vi "configuration UI.vi"() -> ()   [LabVIEW 2013, in "CVT editor node.lvclass"]
uses:
  CVT editor node.lvclass
  <vilib>/NI/Configuration Framework/Node/NodeRef.ctl
  <vilib>/NI/Configuration Framework/Node/NISE_CEF_Node.lvclass
  <vilib>/NI/AMC/Message Queue.ctl
  <vilib>/NI/AMC/Message.ctl
  <vilib>/NI/Tools/Keyed Array/KeyedArray.ctl
  <vilib>/NI/Configuration Framework/Node/UserEventRef.ctl
  <vilib>/NI/Configuration Framework/Controls/EventCluster.ctl
  <vilib>/NI/DCAF UI Toolkit/Controls/Move One Left.ctl
  <vilib>/NI/DCAF UI Toolkit/Controls/Move One Right.ctl
  <vilib>/Utility/miscctls.llb/LVPositionTypeDef.ctl
  <vilib>/Utility/miscctls.llb/LVRowAndColumnTypeDef.ctl
  CVT editor node.lvclass/CVT editor node.ctl
  configuration/CVT configuration.lvclass/CVT configuration.ctl
  <vilib>/NI/Tag Bus Module Framework/channel/channel classification.ctl
  <vilib>/NI/Tag Bus/tag/Data Type.ctl
  <vilib>/NI/Configuration Framework/serializable configuration/NISE_CEF_serializable configuration.lvclass/NISE_CEF_serializable configuration.ctl
  configuration/CVT configuration.lvclass
  <vilib>/NI/Tag Bus/tag/tag descriptor.lvclass/tag descriptor.ctl
  configuration/Write Create Tags_.vi
  <vilib>/Utility/LVClass/Get LV Class Name.vi
  <vilib>/NI/Configuration Framework/error generator/NISE_error generator.vi
  Item Names.vi
  Apply Filter_1D.vi
  Apply Filter_2D.vi
  <vilib>/NI/Module Execution Interface/Engine Configuration/engine configuration.lvclass
  <vilib>/NI/DCAF/Tag Editor Core/Configuration Editor/Classes/Module editor node/module editor node.lvclass
  <vilib>/NI/Configuration Framework/NISE_CEF_TreeControl.lvlib
  <vilib>/NI/Tag Bus/tag/tag descriptor.lvclass
  <vilib>/NI/Tag Bus Module Framework/channel/TBM channel.lvclass
  <vilib>/NI/DCAF/Tag Editor Core/Configuration Editor/Classes/Engine Parent/Engine Parent Editor Node.lvclass
  <vilib>/NI/Configuration Framework/serializable configuration/NISE_CEF_serializable configuration.lvclass
  <vilib>/NI/DCAF UI Toolkit/Controls/DCAF UI Elements.lvlib
  <vilib>/NI/Tools/Keyed Array/Tools_KeyedArray.lvlib
  <vilib>/NI/AMC/AMC.lvlib
panel:
  in  "Top Level Tab Control":enum32{"CVT Channel Mappings"}(tab)
  in  "Create Tags?":bool=TRUE
  in  "Filter":string
  in  "add to":T1
  in  "remove to":T2
  in  "add from":T1
  in  "remove from":T2
  in  "to CVT List":i32(listbox)
  in  "from CVT List":i32(listbox)
  in  "avail tags":i32(listbox)
  in  "Direction":enum32{"From CVT", "To CVT"}(radio)
  in  "user event":T3
  in  "main queue":T4
  in  "node ref":T5
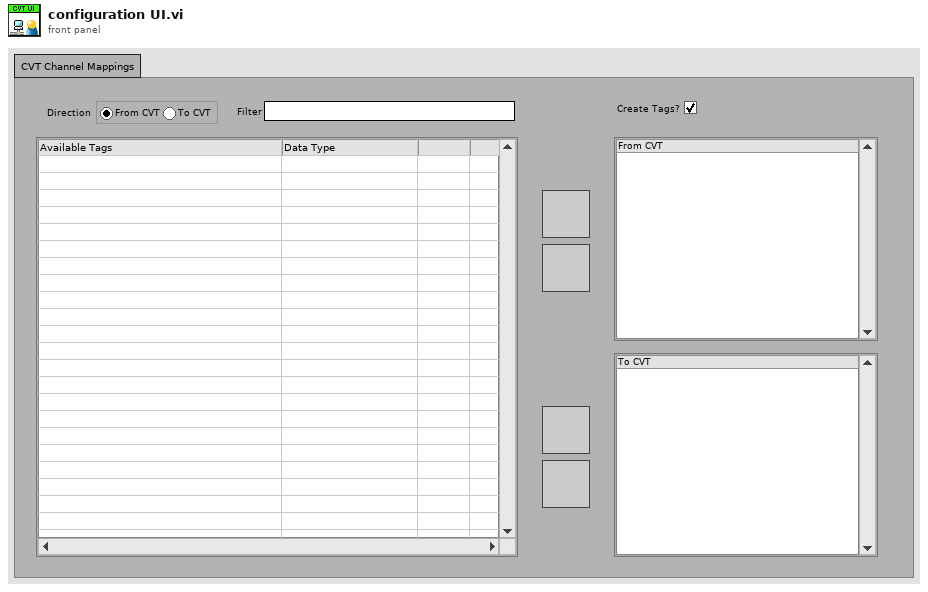
[diagram p1: front panel]
types:
  T1 = typedef "DCAF UI Elements.lvlib/Move One Right.ctl" = bool
  T2 = typedef "DCAF UI Elements.lvlib/Move One Left.ctl" = bool
  T3 = typedef "NISE_CEF_Node.lvclass/UserEventRef.ctl" = refnum<user-event>
  T4 = typedef "AMC.lvlib/Message Queue.ctl" = refnum<queue>
  T5 = typedef "NISE_CEF_Node.lvclass/NodeRef.ctl" = refnum<data-value>
  T6 = typedef "LVPositionTypeDef.ctl" = cluster{"Left":i32, "Top":i32}
  T7 = typedef "NISE_CEF_TreeControl.lvlib/EventCluster.ctl" = cluster{"command":string, "data":string}
  T8 = typedef "LVRowAndColumnTypeDef.ctl" = cluster{"Row":i32, "Column":i32}
  T9 = enum8{"Enabled", "Disabled", "Disabled and Grayed Out"}
  T10 = typedef "tag bus.lvlib/tag descriptor.lvclass/Data Type.ctl" = enum16{"Double", "Single", "I64", "I32", "I16", "I8", "U64", "U32", "U16", "U8", "Boolean", "String", "Array of Double", "Array of Single", "Array of I64", "Array of I32", "Array of I16", "Array of I8", "Array of U64", "Array of U32", "Array of U16", "Array of U8", "Array of Boolean", "Array of String"}
  T11 = typedef "TBM channel.lvclass/channel classification.ctl" = enum16{"input data", "output data", "processing parameter", "processing result"}
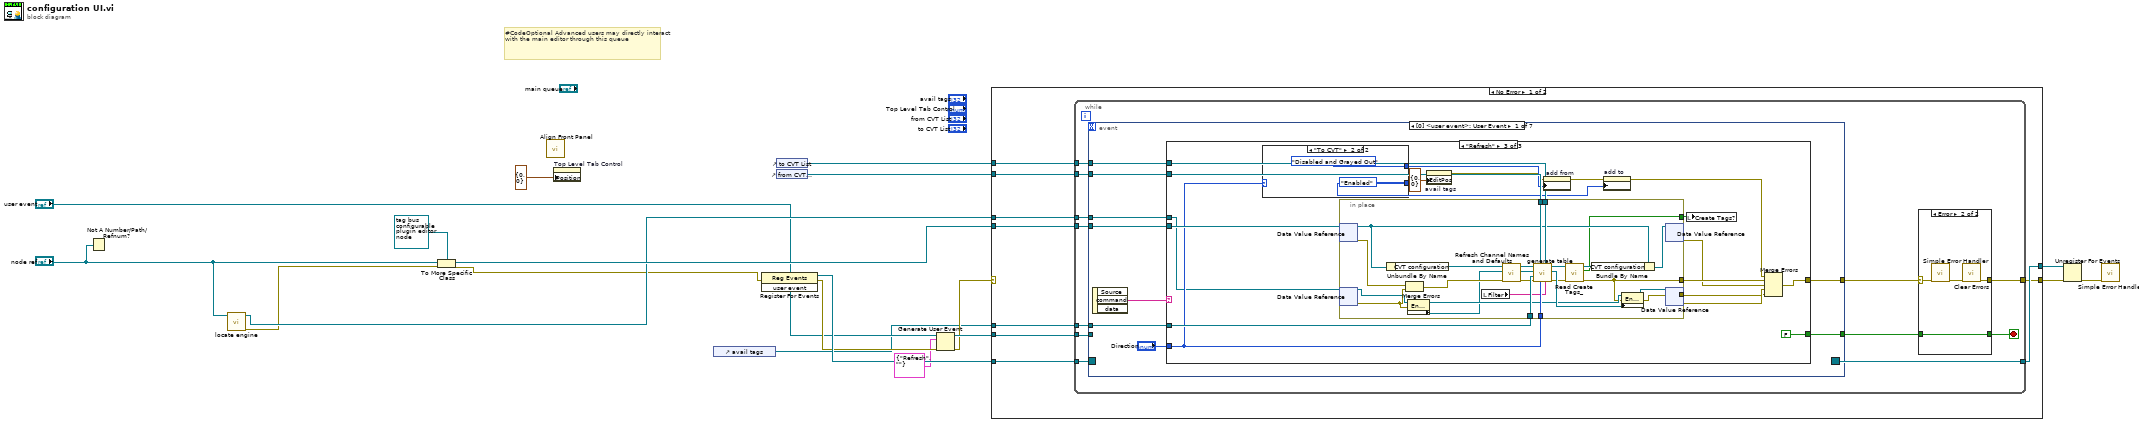
[diagram p0: block diagram]
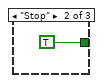
[diagram p4: hidden frame]
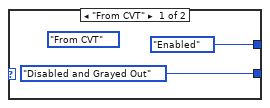
[diagram p5: hidden frame]
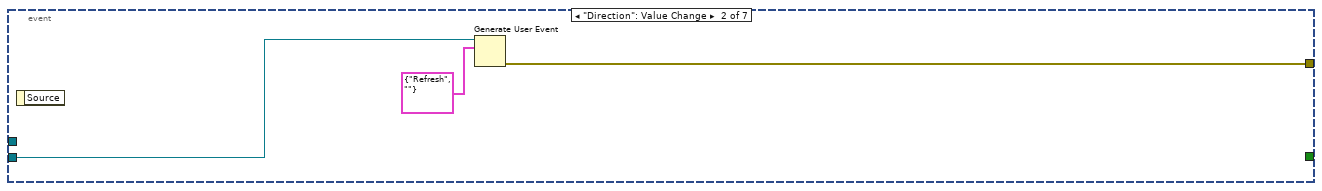
[diagram p6: hidden frame]
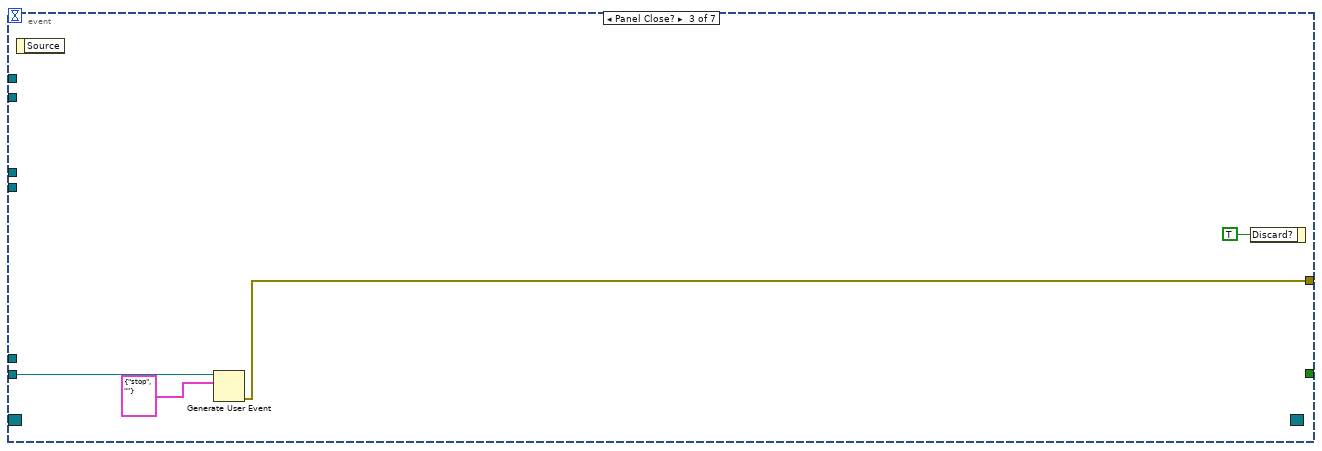
[diagram p7: hidden frame]
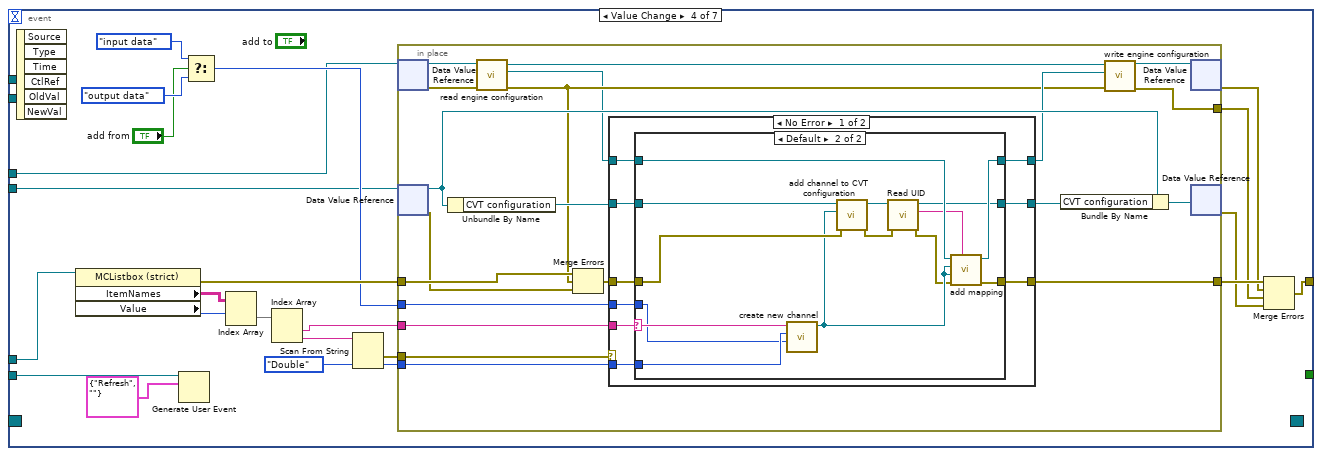
[diagram p8: hidden frame]
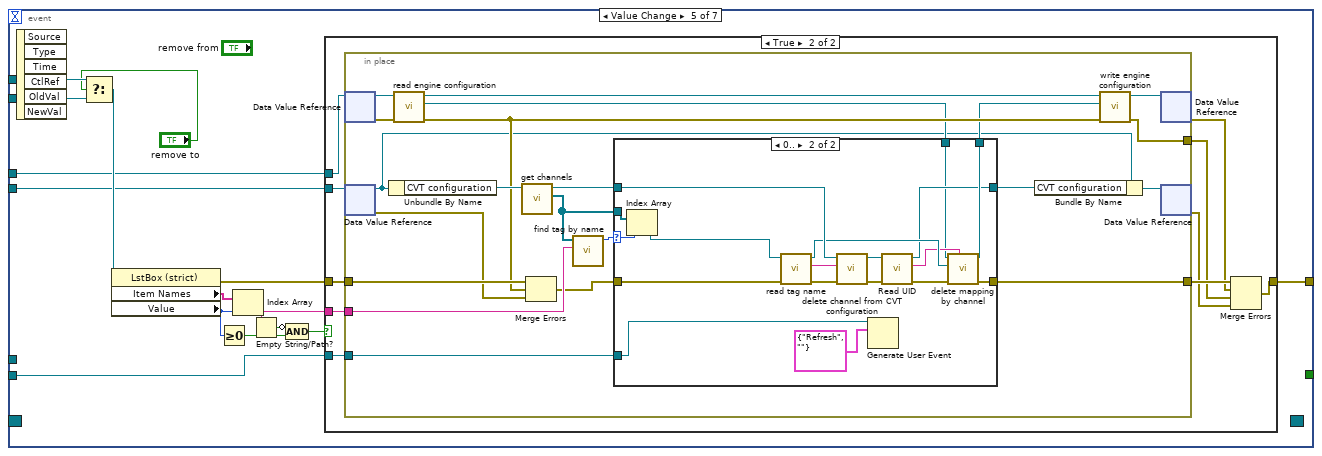
[diagram p11: hidden frame]
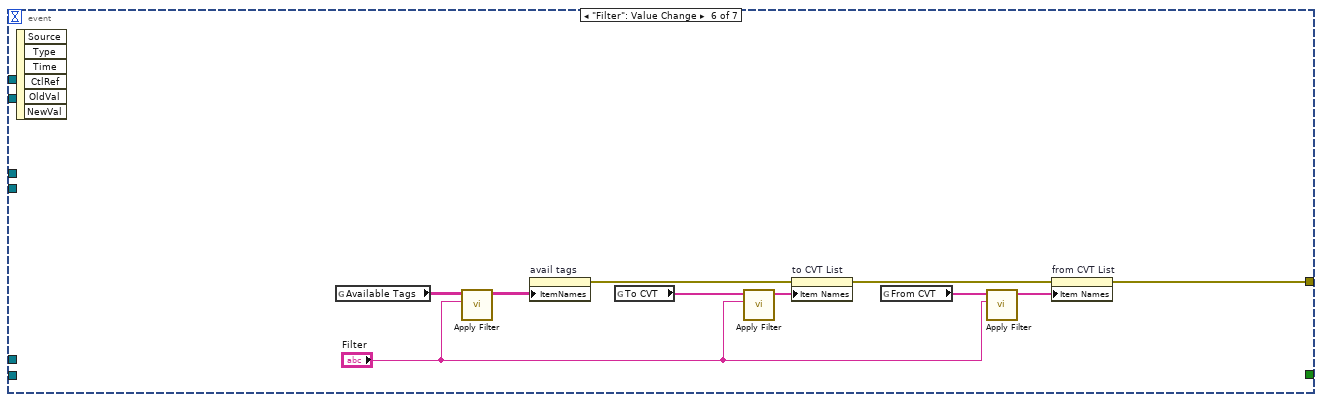
[diagram p14: hidden frame]
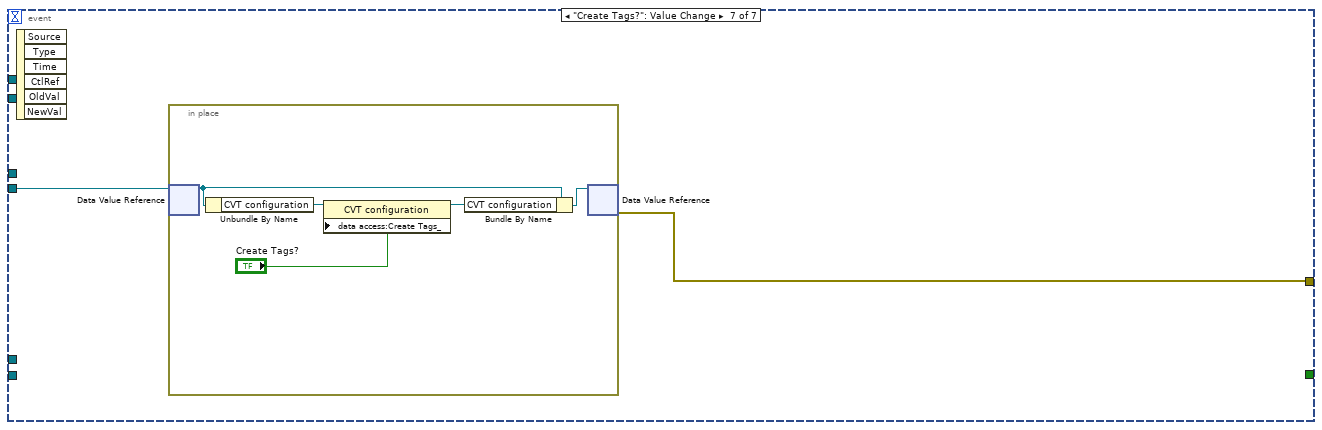
[diagram p15: hidden frame]
diagram:
  # "#CodeOptional Advanced users may directly interact with the main editor through this queue"
  n1 = Not A Number/Path/Refnum?(number/path/refnum="node ref") -> ()  [unwired: 1 out]
  n2 = call <vilib>:"locate engine.vi"("component"="node ref") -> ("error out"=w6:errorcluster, "engine"=w13:refnum<data-value>)  [unwired: 9 in]
  n3 = To More Specific Class(target class=refnum<data-value> refnum ("data value reference"), reference="node ref", error in=w6) -> (specific class reference=w15:refnum<data-value>, error out=w1:errorcluster)
  n4 = call <vilib>:"Align Front Panel.vi"() -> ()  [unwired: 10 in, 2 out]
  n5 = property on="Top Level Tab Control" class="TabCtl (strict)"("Position"=T6 {"Left"=0, "Top"=0}) -> ()  [unwired: 2 in, 2 out]
  n6 = control-ref of="avail tags"() -> (w2:refnum<vi>)
  n7 = register-events(error in=w1, "user event") -> (reference out=w19:refnum<event-registration>, error out=w12:errorcluster)  [unwired: 1 in]
  n8 = control-ref of="to CVT List"() -> (w4:refnum<vi>)
  n9 = control-ref of="from CVT List"() -> (w3:refnum<vi>)
  n10 = Generate User Event(user event="user event", event data cluster=T7 {"command"="Refresh", "data"=""} ("event data"), error in=w12) -> (user event out=w10:T3, error out=w8:errorcluster)  [unwired: 1 in]
  n11 = case shown="No Error" w8 {
    selector: w8 -> [_ w270]
    tunnel: w19 -> [w28 w269]
    tunnel: [w27 w269] -> w18
    tunnel: [w26 w270] -> w17
    tunnel: w15 -> [w25 _]
    tunnel: w13 -> [w24 _]
    tunnel: w2 -> [w23 _]
    tunnel: w4 -> [w22 _]
    tunnel: w3 -> [w21 _]
    tunnel: w10 -> [w20 _]
    frame No Error {
      n12 = while {
        tunnel: w28 -> [w40]
        tunnel: [w39] -> w27
        tunnel: w25 -> [w34]
        tunnel: w24 -> [w33]
        tunnel: w20 -> [w32]
        tunnel: w23 -> [w31]
        tunnel: w22 -> [w30]
        tunnel: w21 -> [w29]
        tunnel: [w35] -> w26
        stop <- w37 stop-if-true
        n13 = event shown="[0] <user event>: User Event" {
          selector: w40 -> [_ _ _ _ _ _ _]
          dyn-events: [_ _ _ _ _ _ _] -> w39
          timeout: _ -> [_ _ _ _ _ _ _]
          tunnel: [w55 _ _ _ _ _ _] -> w36
          tunnel: [w53 w105 w108 w118 w189 w261 w262] -> w38
          tunnel: w34 -> [w52 _ _ w114 w186 _ w263]
          tunnel: w33 -> [w51 _ _ w115 w185 _ _]
          tunnel: w32 -> [_ w106 w109 w133 w188 _ _]
          tunnel: w31 -> [w50 _ _ w128 _ _ _]
          tunnel: w30 -> [w49 _ _ _ w197 _ _]
          tunnel: w29 -> [w48 _ _ _ w198 _ _]
          event User Event {
            n14 = event-data() -> ("command"=w54:string)  [unwired: 1 in, 2 out]
            n15 = case shown="\"Refresh\"" w54 {
              tunnel: [_ TRUE FALSE] -> w55
              tunnel: [_ _ w69] -> w53
              tunnel: w52 -> [_ _ w70]
              tunnel: w51 -> [_ _ w60]
              tunnel: w50 -> [_ _ w73]
              tunnel: w49 -> [_ _ w72]
              tunnel: w48 -> [_ _ w71]
              tunnel: "Direction" -> [_ _ w62]
              frame Default {
              }
              frame "Stop" {
              }
              frame "Refresh" {
                n16 = case shown="\"To CVT\"" w62 {
                  tunnel: [T9."Enabled" ("Disabled") T9."Disabled and Grayed Out" ("Disabled")] -> w66
                  tunnel: [T9."Disabled and Grayed Out" ("Disabled") T9."Enabled" ("Disabled")] -> w65
                  frame "From CVT" {
                    (unwired) enum32{"From CVT", "To CVT"}."From CVT" ("Direction")
                  }
                  frame "To CVT" {
                  }
                }
                n17 = in-place {
                  in-place-border: [w81] -> w74
                  in-place-border: w73 -> [w104]
                  in-place-border: w72 -> [w103]
                  in-place-border: w71 -> [w102]
                  in-place-border: w62 -> [w101]
                  in-place-border: [w93] -> w58
                  in-place-border: [w80] -> w57
                  n18 = in-place-dvr #1(w70) -> (w99:refnum<class "CVT editor node.lvclass">, w100:errorcluster)
                  n19 = in-place-dvr #2(w60) -> (w96:refnum<class "Engine Parent Editor Node.lvclass">, w97:errorcluster)
                  n20 = Unbundle By Name(w99) -> ("CVT configuration"=w89:refnum<class "CVT configuration.lvclass">)
                  n21 = Merge Errors(w100, w97) -> (w91:errorcluster)
                  n22 = property class="Engine Parent Editor Node.lvcla"(reference=w96, error in=w97) -> (reference out=w94:refnum<class "Engine Parent Editor Node.lvclass">, "Data Access:Engine Configuration"=w87:refnum<class "engine configuration.lvclass">)  [unwired: 1 out]
                  n23 = local read "Filter"() -> (w85:string)
                  n24 = call "Refresh Channel Names and Defaults.vi"("error in (no error)"=w91, "engine configuration in"=w87, "CVT configuration in"=w89) -> ("error out"=w90:errorcluster, "engine configuration out"=w86:refnum<class "engine configuration.lvclass">, "CVT configuration out"=w88:refnum<class "CVT configuration.lvclass">)  [unwired: 6 in]
                  n25 = call "generate table.vi"("Filter"=w85, "to cvt"=w103, "Direction"=w101, "from cvt"=w102, "error in"=w90, "avail tags"=w104, "engine configuration in"=w86, "cvt in"=w88) -> ("error out"=w83:errorcluster, "engine configuration out"=w95:refnum<class "engine configuration.lvclass">, "cvt out"=w84:refnum<class "CVT configuration.lvclass">)  [unwired: 1 in]
                  n26 = call "Read Create Tags_.vi"("error in (no error)"=w83, "CVT configuration in"=w84) -> ("error out"=w81:errorcluster, "Create Tags?"=w80:bool, "CVT configuration out"=w82:refnum<class "CVT configuration.lvclass">)  [unwired: 7 in]
                  n27 = Bundle By Name(cluster=w99, "CVT configuration"=w82) -> (w98:refnum<class "CVT editor node.lvclass">)
                  n28 = property class="Engine Parent Editor Node.lvcla"(reference=w94, error in=w81, "Data Access:Engine Configuration"=w95) -> (reference out=w92:refnum<class "Engine Parent Editor Node.lvclass">, error out=w93:errorcluster)
                  n29 = in-place-dvr #1(w98) -> (w68:errorcluster)  [unwired: 1 out]
                  n30 = in-place-dvr #2(w92) -> (w59:errorcluster)  [unwired: 1 out]
                }
                n31 = property on="avail tags" class="MCListbox (strict)"("EditPos"=T8 {"Row"=0, "Column"=0} ("Edit Position")) -> (error out=w63:errorcluster)  [unwired: 2 in, 1 out]
                n32 = property on="add from" class="Bool"(error in=w63, "DisabledEnum"=w66) -> (error out=w67:errorcluster)  [unwired: 1 in, 1 out]
                n33 = property on="add to" class="Bool"(error in=w67, "DisabledEnum"=w65) -> (error out=w61:errorcluster)  [unwired: 1 in, 1 out]
                n34 = local write "Create Tags?"(w57) -> ()
                n35 = Merge Errors(w61, w74, w68, w59, w58) -> (w69:errorcluster)
              }
            }
          }
          event "Direction": Value Change {
            n36 = event-data() -> ()  [unwired: 1 in, 1 out]
            n37 = Generate User Event(user event=w106, event data cluster=T7 {"command"="Refresh", "data"=""} ("event data")) -> (error out=w105:errorcluster)  [unwired: 2 in, 1 out]
          }
          event Panel Close? {
            n38 = event-data() -> ()  [unwired: 1 in, 1 out]
            n39 = Generate User Event(user event=w109, event data cluster=T7 {"command"="stop", "data"=""} ("event data")) -> (error out=w108:errorcluster)  [unwired: 2 in, 1 out]
            n40 = event-data("Discard?"=TRUE) -> ()  [unwired: 1 in, 1 out]
          }
          event Value Change {
            n41 = event-data() -> ()  [unwired: 1 in, 6 out]
            n42 = property class="MCListbox (strict)"(reference=w128) -> (error out=w129:errorcluster, "ItemNames"=w127:string[][], "Value"=w126:i32)  [unwired: 1 in, 1 out]
            n43 = Generate User Event(user event=w133, event data cluster=T7 {"command"="Refresh", "data"=""} ("event data")) -> ()  [unwired: 2 in, 2 out]
            n44 = Select(t=channel_classification."input data" ("channel classification"), s="add from", f=channel_classification."output data" ("channel classification")) -> (s? t:f=w119:T11)
            n45 = Index Array(array=w127, index (row)=w126) -> (element=w123:string[])  [unwired: 1 in]
            n46 = Index Array(array=w123) -> (element #1=w122:string, element #2=w125:string)  [unwired: 2 in]
            n47 = Scan From String(input string=w125, default 1=Data_Type."Double" ("data type")) -> (error out=w121:errorcluster, output 1=w120:T10)  [unwired: 3 in, 2 out]
            n48 = in-place {
              in-place-border: [w154] -> w134
              in-place-border: w129 -> [w153]
              in-place-border: w122 -> [w152]
              in-place-border: w121 -> [w151]
              in-place-border: w120 -> [w150]
              in-place-border: w119 -> [w149]
              in-place-border: [w139] -> w113
              n49 = in-place-dvr #3(w115) -> (w142:refnum<class "Engine Parent Editor Node.lvclass">, w137:errorcluster)
              n50 = in-place-dvr #4(w114) -> (w145:refnum<class "CVT editor node.lvclass">, w143:errorcluster)
              n51 = Unbundle By Name(w145) -> ("CVT configuration"=w147:refnum<class "CVT configuration.lvclass">)
              n52 = call <vilib>:"read engine configuration.vi"("error in"=w137, "Engine Parent Editor Node in"=w142) -> ("error out"=w136:errorcluster, "engine configuration"=w135:refnum<class "engine configuration.lvclass">, "Engine Parent Editor Node out"=w138:refnum<class "Engine Parent Editor Node.lvclass">)  [unwired: 7 in]
              n53 = Merge Errors(w153, w136, w143) -> (w148:errorcluster)
              n54 = case shown="No Error" w151 {
                tunnel: [w163 w181] -> w154
                tunnel: [w162 w183] -> w140
                tunnel: [w161 w182] -> w146
                tunnel: w147 -> [w160 w182]
                tunnel: w135 -> [w159 w183]
                tunnel: w148 -> [w158 w181]
                tunnel: w152 -> [w157 _]
                tunnel: w150 -> [w156 _]
                tunnel: w149 -> [w155 _]
                frame No Error {
                  n55 = case shown="Default" w157 {
                    selector: w157 -> [_ w174]
                    tunnel: [w166 w180] -> w163
                    tunnel: w158 -> [w166 w176]
                    tunnel: w159 -> [w164 w179]
                    tunnel: [w165 w168] -> w161
                    tunnel: w160 -> [w165 w177]
                    tunnel: [w164 w178] -> w162
                    tunnel: w156 -> [_ w173]
                    tunnel: w155 -> [_ w172]
                    frame "" {
                    }
                    frame Default {
                      n56 = call <vilib>:"create new channel.vi"("channel classification"=w172, "data type"=w173, "channel name"=w174) -> ("channel"=w171:refnum<class "TBM channel.lvclass">)  [unwired: 8 in]
                      n57 = call "add channel to CVT configuration.vi"("error in"=w176, "channel"=w171, "CVT configuration in"=w177) -> ("error out"=w175:errorcluster, "CVT configuration out"=w169:refnum<class "CVT configuration.lvclass">)  [unwired: 7 in]
                      n58 = call <vilib>:"Read UID.vi"("error in"=w175, "configuration in"=w169) -> ("error out"=w170:errorcluster, "instance id"=w167:string, "configuration out"=w168:refnum<class "CVT configuration.lvclass">)  [unwired: 7 in]
                      n59 = call <vilib>:"add mapping.vi"("owner ID"=w167, "error in"=w170, "channel"=w171, "tag descriptor"=w171, "engine configuration"=w179) -> ("error out"=w180:errorcluster, "engine configuration out"=w178:refnum<class "engine configuration.lvclass">)  [unwired: 5 in]
                    }
                  }
                }
                frame Error {
                }
              }
              n60 = Bundle By Name(cluster=w145, "CVT configuration"=w146) -> (w144:refnum<class "CVT editor node.lvclass">)
              n61 = call <vilib>:"write engine configuration.vi"("error in"=w136, "engine configuration"=w140, "Engine Parent Editor Node in"=w138) -> ("error out"=w139:errorcluster, "Engine Parent Editor Node out"=w141:refnum<class "Engine Parent Editor Node.lvclass">)  [unwired: 7 in]
              n62 = in-place-dvr #3(w141) -> (w117:errorcluster)  [unwired: 1 out]
              n63 = in-place-dvr #4(w144) -> (w116:errorcluster)  [unwired: 1 out]
            }
            n64 = Merge Errors(w134, w117, w113, w116) -> (w118:errorcluster)
          }
          event Value Change {
            n65 = event-data() -> ()  [unwired: 1 in, 6 out]
            n66 = Select(t=w197, s="remove to", f=w198) -> (s? t:f=w196:refnum<vi>)
            n67 = property class="LstBox (strict)"(reference=w196) -> (error out=w190:errorcluster, "Item Names"=w195:string[], "Value"=w194:i32)  [unwired: 1 in, 1 out]
            n68 = Greater Or Equal To 0?(x=w194) -> (x >= 0?=w192:bool)
            n69 = Index Array(array=w195, index=w194) -> (element=w187:string)
            n70 = Empty String/Path?(string/path=w187) -> (empty?=w193:bool)
            n71 = Compound Arithmetic op=AND(invert w193, w192) -> (w191:bool)
            n72 = case shown="True" w191 {
              tunnel: w190 -> [w199 w206]
              tunnel: [w199 w205] -> w189
              tunnel: w188 -> [_ w209]
              tunnel: w187 -> [_ w208]
              tunnel: w186 -> [_ w204]
              tunnel: w185 -> [_ w203]
              frame False {
              }
              frame True {
                n73 = in-place {
                  in-place-border: w209 -> [w230]
                  in-place-border: w208 -> [w229]
                  in-place-border: [w226] -> w207
                  in-place-border: w206 -> [w225]
                  in-place-border: [w219] -> w200
                  n74 = in-place-dvr #5(w203) -> (w222:refnum<class "Engine Parent Editor Node.lvclass">, w217:errorcluster)
                  n75 = in-place-dvr #6(w204) -> (w212:refnum<class "CVT editor node.lvclass">, w216:errorcluster)
                  n76 = Unbundle By Name(w212) -> ("CVT configuration"=w218:refnum<class "CVT configuration.lvclass">)
                  n77 = call <vilib>:"read engine configuration.vi"("error in"=w217, "Engine Parent Editor Node in"=w222) -> ("error out"=w215:errorcluster, "engine configuration"=w214:refnum<class "engine configuration.lvclass">, "Engine Parent Editor Node out"=w221:refnum<class "Engine Parent Editor Node.lvclass">)  [unwired: 7 in]
                  n78 = call-dynamic "get channels.vi"("CVT configuration in"=w218) -> ("channels"=w224:refnum<class "TBM channel.lvclass">[], "CVT configuration out"=w227:refnum<class "CVT configuration.lvclass">)  [unwired: 9 in]
                  n79 = Merge Errors(w225, w215, w216) -> (w223:errorcluster)
                  n80 = call <vilib>:"find tag by name.vi"("name"=w229, "tags in"=w224) -> ("index"=w228:i32)  [unwired: 9 in]
                  n81 = case shown="0.." w228 {
                    selector: w228 -> [_ w249]
                    tunnel: w230 -> [_ w250]
                    tunnel: w227 -> [w233 w247]
                    tunnel: [w233 w236] -> w210
                    tunnel: [w232 w243] -> w226
                    tunnel: w223 -> [w232 w246]
                    tunnel: [w231 w244] -> w213
                    tunnel: w224 -> [_ w248]
                    tunnel: w214 -> [w231 w234]
                    frame ..-1 {
                    }
                    frame 0.. {
                      n82 = Index Array(array=w248, index=w249) -> (element=w241:refnum<class "TBM channel.lvclass">)
                      n83 = call <vilib>:"read tag name.vi"("error in"=w246, "system tag in"=w241) -> ("error out"=w242:errorcluster, "name"=w239:string, "system tag out"=w240:refnum<class "TBM channel.lvclass">)  [unwired: 7 in]
                      n84 = call "delete channel from CVT configuration.vi"("error in"=w242, "channel to delete"=w239, "CVT configuration in"=w247) -> ("error out"=w245:errorcluster, "CVT configuration out"=w237:refnum<class "CVT configuration.lvclass">)  [unwired: 7 in]
                      n85 = Generate User Event(user event=w250, event data cluster=T7 {"command"="Refresh", "data"=""} ("event data")) -> ()  [unwired: 2 in, 2 out]
                      n86 = call <vilib>:"Read UID.vi"("error in"=w245, "configuration in"=w237) -> ("error out"=w238:errorcluster, "instance id"=w235:string, "configuration out"=w236:refnum<class "CVT configuration.lvclass">)  [unwired: 7 in]
                      n87 = call <vilib>:"delete mapping by channel.vi"("owner ID"=w235, "error in"=w238, "channel"=w240, "engine configuration in"=w234) -> ("error out"=w243:errorcluster, "engine configuration out"=w244:refnum<class "engine configuration.lvclass">)  [unwired: 6 in]
                    }
                  }
                  n88 = Bundle By Name(cluster=w212, "CVT configuration"=w210) -> (w211:refnum<class "CVT editor node.lvclass">)
                  n89 = call <vilib>:"write engine configuration.vi"("error in"=w215, "engine configuration"=w213, "Engine Parent Editor Node in"=w221) -> ("error out"=w219:errorcluster, "Engine Parent Editor Node out"=w220:refnum<class "Engine Parent Editor Node.lvclass">)  [unwired: 7 in]
                  n90 = in-place-dvr #5(w220) -> (w202:errorcluster)  [unwired: 1 out]
                  n91 = in-place-dvr #6(w211) -> (w201:errorcluster)  [unwired: 1 out]
                }
                n92 = Merge Errors(w207, w202, w200, w201) -> (w205:errorcluster)
              }
            }
          }
          event "Filter": Value Change {
            n93 = event-data() -> ()  [unwired: 1 in, 6 out]
            n94 = global read "Item Names.vi" "Available Tags"() -> (w254:string[][])
            n95 = call-poly "Apply Filter.vi"("Filter"="Filter", "Item names"=w254) -> ("Filtered Item Names"=w253:string[][])  [unwired: 9 in]
            n96 = property on="avail tags" class="MCListbox (strict)"("ItemNames"=w253) -> (error out=w255:errorcluster)  [unwired: 2 in, 1 out]
            n97 = global read "Item Names.vi" "To CVT"() -> (w256:string[])
            n98 = call-poly "Apply Filter.vi"("Filter"="Filter", "Item names"=w256) -> ("Filtered Item Names"=w257:string[])  [unwired: 9 in]
            n99 = property on="to CVT List" class="LstBox (strict)"(error in=w255, "Item Names"=w257) -> (error out=w258:errorcluster)  [unwired: 1 in, 1 out]
            n100 = global read "Item Names.vi" "From CVT"() -> (w260:string[])
            n101 = call-poly "Apply Filter.vi"("Filter"="Filter", "Item names"=w260) -> ("Filtered Item Names"=w259:string[])  [unwired: 9 in]
            n102 = property on="from CVT List" class="LstBox (strict)"(error in=w258, "Item Names"=w259) -> (error out=w261:errorcluster)  [unwired: 1 in, 1 out]
          }
          event "Create Tags?": Value Change {
            n103 = event-data() -> ()  [unwired: 1 in, 6 out]
            n104 = in-place {
              n105 = in-place-dvr #7(w263) -> (w268:refnum<class "CVT editor node.lvclass">)  [unwired: 1 out]
              n106 = Unbundle By Name(w268) -> ("CVT configuration"=w266:refnum<class "CVT configuration.lvclass">)
              n107 = property class="CVT configuration"(reference=w266, "data access:Create Tags_"="Create Tags?") -> (reference out=w265:refnum<class "CVT configuration.lvclass">)  [unwired: 1 in, 1 out]
              n108 = Bundle By Name(cluster=w268, "CVT configuration"=w265) -> (w267:refnum<class "CVT editor node.lvclass">)
              n109 = in-place-dvr #7(w267) -> (w262:errorcluster)  [unwired: 1 out]
            }
          }
        }
        n110 = case shown="Error" w38 {
          selector: w38 -> [w41 w45]
          tunnel: [w42 w46] -> w37
          tunnel: w36 -> [w42 w46]
          tunnel: [w41 w43] -> w35
          frame No Error {
          }
          frame Error {
            n111 = call <vilib>:"Simple Error Handler.vi"("error in (no error)"=w45) -> ("error out"=w44:errorcluster)  [unwired: 4 in, 4 out]
            n112 = call <vilib>:"Clear Errors.vi"("error in (no error)"=w44) -> ("error out"=w43:errorcluster)  [unwired: 6 in]
          }
        }
      }
    }
    frame Error {
    }
  }
  n113 = Unregister For Events(event registration refnum=w18, error in=w17) -> (error out=w14:errorcluster)
  n114 = call <vilib>:"Simple Error Handler.vi"("error in (no error)"=w14) -> ()  [unwired: 4 in, 5 out]
